vi "New.vi"(8 "error in (no error)":errorcluster, 10 "Parent":refnum<class "Config Element.lvclass">, 11 "Name":string) -> (0 "error out":errorcluster, 2 "Config Element":refnum<class "Config Element.lvclass">, 3 "Cluster out":refnum<class "Cluster Config.lvclass">)   [LabVIEW 2020, in "VolatusConfig.lvlib" / "Cluster Config.lvclass"]
uses:
  Cluster Config.lvclass
  C:/dev/lv20CE/relink/lv-volatus/VolatusConfig/VolatusConfigElement/VolatusConfigElement.lvclass
  lv-cdm/CDM-Config/Config Element/Config Element.lvclass
  Meta Type.ctl
  lv-cdm/CDM-Config/Value Type.ctl
  Cluster Config.lvclass/Cluster Config.ctl
  lv-cdm/CDM-Config/CDM-Config.lvlib
  VolatusConfigElement/VolatusConfigElement.lvclass
  VolatusConfig.lvlib
  C:/dev/lv20CE/relink/lv-volatus/VolatusConfig/Cluster/Cluster Config.lvclass
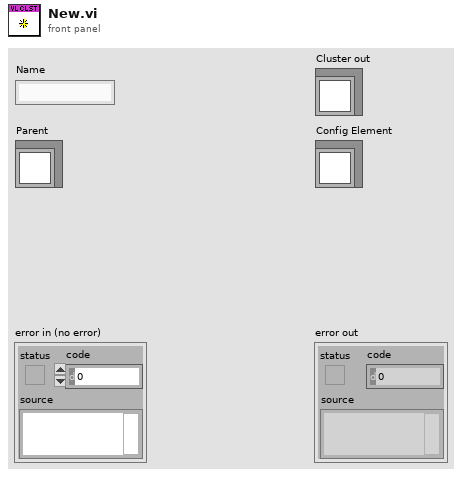
[diagram p1: front panel]
types:
  T1 = typedef "CDM-Config.lvlib/Value Type.ctl" = enum16{"String", "Number", "Bool", "Object", "Array"}
  T2 = typedef "VolatusConfig.lvlib/Meta Type.ctl" = enum16{"UNKNOWN", "VL_System", "VL_Cluster", "VL_Node", "VL_Task", "VL_Group", "VL_Channel", "VL_Task_List", "VL_Scaling", "VL_Sensor", "VL_Sensor_List", "VL_Scale"}
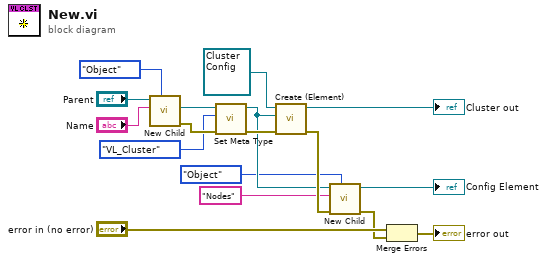
[diagram p0: block diagram]
diagram:
  n1 = call "New Child.vi"("Value Type (Object)"=Value_Type."Object" ("Value Type (String)"), "Child Name"="Name", "Config Element in"="Parent") -> ("error out"=w16:errorcluster, "New Child"=w11:refnum<class "Config Element.lvclass">)  [unwired: 6 in, 1 out]
  n2 = call "Set Meta Type.vi"("error in (no error)"=w16, "Meta Type"=Meta_Type."VL_Cluster", "Element In"=w11) -> ("error out"=w9:errorcluster, "Element"=w5:refnum<class "Config Element.lvclass">)  [unwired: 7 in]
  n3 = call "Create (Element).vi"("error in (no error)"=w9, "Element"=w5, "VolatusConfigElement in"=refnum<class "Cluster Config.lvclass"> refnum ("Cluster in")) -> ("error out"=w17:errorcluster, "VolatusConfigElement out"=→"Cluster out":refnum<class "Cluster Config.lvclass">)  [unwired: 7 in]
  n4 = call "New Child.vi"("Value Type (Object)"=Value_Type."Object" ("Value Type (String)"), "error in (no error)"=w17, "Child Name"="Nodes", "Config Element in"=w5) -> ("error out"=w2:errorcluster, "Config Element out"=→"Config Element":refnum<class "Config Element.lvclass">)  [unwired: 5 in, 1 out]
  n5 = Merge Errors("error in (no error)", w2) -> (→"error out":errorcluster)
